vi "Build CE Deploy - Can VI have Call Library Node.vi"(10 "default relative path to DLL":path=path "../../cersrc/celveng*.dll", 11 "VI Path":path) -> (0 "Can have CLN":bool, 2 "celveng*.dll path relative to VI":path)   [LabVIEW 2021]
doc: "::: CalcExpress Toolkit :::\nCopyright (c) 2000-2026 Konstantin Shifershteyn. All rights reserved."
uses:
  <vilib>/Utility/lvfile.llb/FT_FileTypes.ctl
  <vilib>/Utility/lvfile.llb/NI_FileType.lvlib
panel:
  # "CalcExpress Toolkit\nCopyright (c) 2000-2026 Konstantin Shifershteyn"
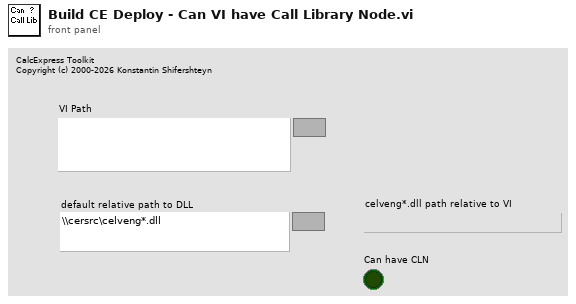
[diagram p1: front panel]
types:
  T1 = typedef "NI_FileType.lvlib/FT_FileTypes.ctl" = enum32{"Invalid file/path", "Unknown type", "Instrument", "Control", "Polymorphic VI", "Project", "Library", "LVClass", "XControl", "XNode", "CIN", "Run-time menu", "Palette menu", "LLB", "Shortcut", "Directory", "Class Private Data Control", "Statechart", "MathScript .m file", "Ladder Diagram", "LVLibp"}
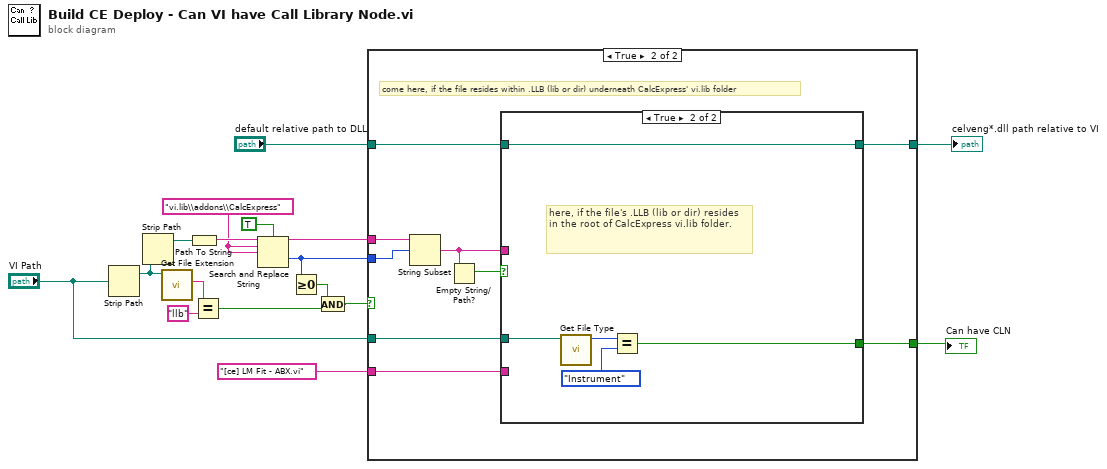
[diagram p0: block diagram]
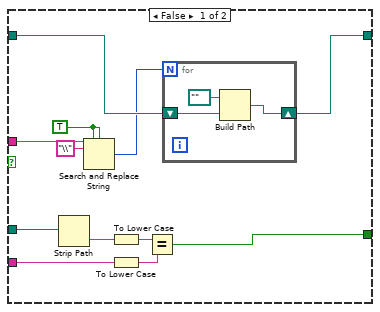
[diagram p3: hidden frame]
diagram:
  w8 = "vi.lib\\addons\\CalcExpress"
  n1 = Strip Path(path="VI Path") -> (stripped path=w13:path)  [unwired: 1 out]
  n2 = Strip Path(path=w13) -> (stripped path=w14:path)  [unwired: 1 out]
  n3 = call <vilib>:"Get File Extension.vi"("file"=w13) -> ("lowercase file extension"=w17:string)  [unwired: 6 in, 4 out]
  n4 = Path To String(path=w14) -> (string=w15:string)
  n5 = Equal?(x=w17, y="llb") -> (x = y?=w12:bool)
  n6 = Search and Replace String(case sensitive?=TRUE, input string=w15, search string=w8, replace string=w8) -> (result string=w7:string, offset past replacement=w6:i32)  [unwired: 4 in, 2 out]
  n7 = Greater Or Equal To 0?(x=w6) -> (x >= 0?=w9:bool)
  n8 = And(x=w9, y=w12) -> (x .and. y?=w10:bool)
  n9 = case shown="True" w10 {
    tunnel: w7 -> [_ w27]
    tunnel: w6 -> [_ w26]
    tunnel: "VI Path" -> [_ w25]
    tunnel: [_ w24] -> w4
    tunnel: "[ce] LM Fit - ABX.vi" -> [_ w22]
    tunnel: [w18 w21] -> w2
    tunnel: "default relative path to DLL" -> [w18 w20]
    frame False {
    }
    frame True {
      # "come here, if the file resides within .LLB (lib or dir) underneath CalcExpress' vi.lib folder"
      n10 = String Subset(string=w27, offset (0)=w26) -> (substring=w19:string)  [unwired: 1 in]
      n11 = Empty String/Path?(string/path=w19) -> (empty?=w23:bool)
      n12 = case shown="True" w23 {
        tunnel: w25 -> [w37 w45]
        tunnel: [w35 w44] -> w24
        tunnel: w22 -> [w34 _]
        tunnel: [w29 w43] -> w21
        tunnel: w20 -> [w30 w43]
        tunnel: w19 -> [w33 _]
        frame False {
          w31 = TRUE
          n13 = Strip Path(path=w37) -> (name=w36:string)  [unwired: 1 out]
          n14 = Search and Replace String(replace all?=w31, case sensitive?=w31, input string=w33, search string="\\") -> (number of replacements=w28:i32)  [unwired: 4 in, 3 out]
          n15 = To Lower Case(string=w36) -> (all lower case string=w39:string)
          n16 = To Lower Case(string=w34) -> (all lower case string=w38:string)
          n17 = Equal?(x=w39, y=w38) -> (x = y?=w35:bool)
          n18 = for {
            N: w28 -> [_]
            shift-right: [w41] -> w29
            shift-left: w30 -> [w42]
            n19 = Build Path(base path=path "..", name or relative path=w42) -> (appended path=w41:path)
          }
        }
        frame True {
          # "here, if the file's .LLB (lib or dir) resides in the root of CalcExpress vi.lib folder."
          n20 = call <vilib>:"Get File Type.vi"("path"=w45) -> ("file type"=w47:T1)  [unwired: 8 in, 2 out]
          n21 = Equal?(x=w47, y=FT_FileTypes."Instrument" ("file type")) -> (x = y?=w44:bool)
        }
      }
    }
  }
  "Can have CLN" <- w4
  "celveng*.dll path relative to VI" <- w2
